vi "XYPlotterUI.vi"() -> ()   [LabVIEW 2025, in "XY Plotter.lvlib" / "XY Plotter.lvclass"]
uses:
  XY Plotter.lvclass
  Users/Public/Documents/Sandia National Labs/TSS Plugin/CEF.lvlibp/Node/mainQref.ctl
  Users/Public/Documents/Sandia National Labs/TSS Plugin/CEF.lvlibp/Node/UserEventRef.ctl
  XY Plotter configuration/XY Plotter.ctl
  Users/Public/Documents/Sandia National Labs/TSS Plugin/CEF.lvlibp/Node/NodeRef.ctl
  Users/Public/Documents/Sandia National Labs/TSS Plugin/CEF.lvlibp/Node/CEF_Node.lvclass
  XY Plotter.lvclass/XY Plotter.ctl
  XY Plotter configuration/XY Plotter configuration.lvclass/XY Plotter configuration.ctl
  <vilib>/Utility/miscctls.llb/LVAnnotationListTypeDef.ctl
  XY Plotter configuration/Read XY Plotter.vi
  XY Plotter configuration/Write XY Plotter.vi
  <vilib>/Analysis/baseanly.llb/Mean (DBL).vi
  C:/Users/Public/Documents/Sandia National Labs/TSS Plugin/CEF.lvlibp/serializable node/CEF_serializable node.lvclass
  C:/Users/Public/Documents/Sandia National Labs/TSS Plugin/CEF.lvlibp/Node/CEF_Node.lvclass
  C:/Working copy/TS Manager/Plugin/Special Test/XY Plotter/XY  Plotter/XY Plotter.lvclass
  <vilib>/Analysis/NI_AALBase.lvlib
  XY Plotter configuration/XY Plotter configuration.lvclass
panel:
  in  "node ref":T1
  in  "XY Plotter Setting":T2={"Data Rate"=100, "Y-Scales"=[{"Label"="Amplitude", "Max"=5.0, "Min"=-5.0, "Unit"=enum."V", "Visible"=TRUE}, {"Label"="", "Max"=100.0, "Min"=-100.0, "Unit"=enum."V", "Visible"=TRUE}], "Note"="", "History Length"=5, "DataLog Path"=path "C:/_Data_Log", "Plot type"=FALSE, "X-Scales"=[{"Label"="Amplitude", "Max"=5.0, "Min"=-5.0, "Unit"=enum."in", "Visible"=TRUE}, {"Label"="", "Max"=100.0, "Min"=-100.0, "Unit"=enum."---", "Visible"=TRUE}], "Plot List"=[{"Plot Name"="Ch1", "X Scale Index"=0, "Y Scale Index"=0, "Visible"=TRUE}, {"Plot Name"="Ch1", "X Scale Index"=0, "Y Scale Index"=0, "Visible"=TRUE}]}
  in  "main queue":T3
  in  "user event":T4
  out "Note":string="ASDFASD\nASDFASD\nF\nASDF\nA\nSDF"
  in  "XY Plot":cluster{"Wavenumber":dbl[], "Data":dbl[]}[](graph)
  in  "Running":bool
  in  "Snap plot":u16(ring)=1 items=["Ch1", "Ch1"]
  in  "Cursor":bool caption="Draw"
  out "Live Loop":u32 caption="ms"
  in  "Settings":bool
  in  "P/N :":string="1D8674-P0100" caption="live data"
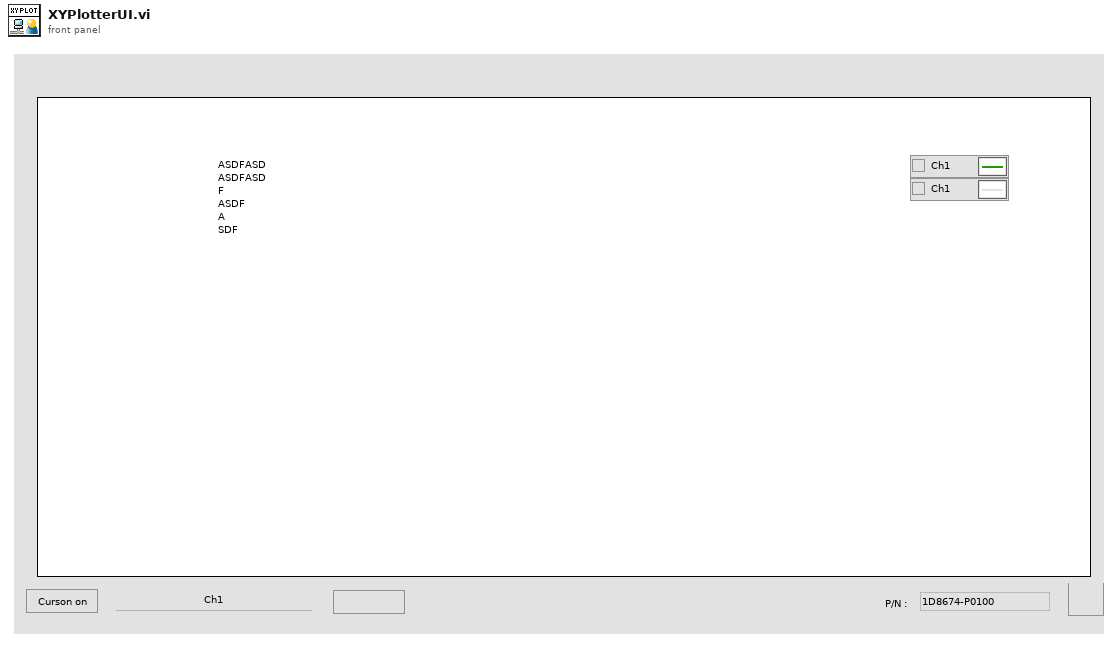
[diagram p1: front panel]
types:
  T1 = typedef "CEF.lvlibp/CEF_Node.lvclass/NodeRef.ctl" = refnum<data-value>
  T2 = typedef "XY Plotter.lvlib/XY Plotter configuration.lvclass/XY Plotter.ctl" = cluster{"Data Rate":i32, "Y-Scales":cluster{"Label":string, "Max":dbl, "Min":dbl, "Unit":enum16{"---", "V", "mA", "sec", "dB", "deg", "in/s", "in", "lbf", "Hz", "psi", "gpm"}, "Visible":bool}[], "Note":string, "History Length":i32, "DataLog Path":path, "Plot type":bool, "X-Scales":cluster{"Label":string, "Max":dbl, "Min":dbl, "Unit":enum16{"---", "V", "mA", "sec", "dB", "deg", "in/s", "in", "lbf", "Hz", "psi", "gpm"}, "Visible":bool}[], "Plot List":cluster{"Plot Name":string, "X Scale Index":u32, "Y Scale Index":u32, "Visible":bool}[]}
  T3 = typedef "CEF.lvlibp/CEF_Node.lvclass/mainQref.ctl" = refnum<queue>
  T4 = typedef "CEF.lvlibp/CEF_Node.lvclass/UserEventRef.ctl" = refnum<user-event>
  T5 = cluster{"XY Plot":refnum<vi>, "Snap plot":refnum<vi>}
  T6 = enum8{"Enabled", "Disabled", "Disabled and Grayed Out"}
  T7 = typedef "LVAnnotationListTypeDef.ctl" = cluster{"Name":string, "Color":u32, "Style":u8, "Point Style":u8, "Name Visible":bool, "Allow Drag":bool, "Annotation Mode":u32, "Plot":i32, "Index":i32, "Position":cluster{"X":dbl, "Y":dbl}, "X Scale":u32, "Y Scale":u32, "Show Arrow":bool, "Lock Name":bool, "Plot Area":i32, "Label Offset":cluster{"X":dbl, "Y":dbl}}[]
  T8 = cluster{"XY Plot":refnum<vi>, "XY Plotter Setting":refnum<vi>, "CursRef":refnum<vi>}
  T9 = typedef "LVPoint32TypeDef.ctl" = cluster{"Horizontal":i32, "Vertical":i32}
  T10 = typedef "LVCursorListTypeDef.ctl" = cluster{"Name":string, "Color":u32, "Style":u8, "Point Style":u8, "Name Visible":bool, "Allow Drag":bool, "Cursor Mode":u32, "Plot":i32, "Index":i32, "Position":cluster{"X":dbl, "Y":dbl}, "X Scale":u32, "Y Scale":u32, "Watch Plots":i32[], "Watch All Plots":bool, "Plot Area":i32, "Label Offset":cluster{"X":dbl, "Y":dbl}}[]
  T11 = cluster{"Plot Name":string, "X Scale Index":u32, "Y Scale Index":u32, "Visible":bool}[]
  T12 = cluster{"Name":string, "Color":u32, "Style":u8, "Point Style":u8, "Name Visible":bool, "Allow Drag":bool, "Annotation Mode":u32, "Plot":i32, "Index":i32, "Position":cluster{"X":dbl, "Y":dbl}, "X Scale":u32, "Y Scale":u32, "Show Arrow":bool, "Lock Name":bool, "Plot Area":i32, "Label Offset":cluster{"X":dbl, "Y":dbl}}
  T13 = cluster{"Shift":bool, "Ctrl":bool, "Alt":bool, "Cmd":bool, "Opt":bool}
  T14 = typedef "eventvkey.ctl" = enum16{"ASCII", "Enter", "Return", "Shift", "Ctrl", "Alt", "Cmd", "Opt", "Caps", "NumLock", "Clear", "Break", "Up", "Down", "Left", "Right", "Insert", "Delete", "Home", "End", "PageUp", "PageDown", "Escape", "Help", "Pause", "ScrollLock", "F1", "F2", "F3", "F4", "F5", "F6", "F7", "F8", "F9", "F10", "F11", "F12", "F13", "F14", "F15", "F16", "F17", "F18", "F19", "F20", "F21", "F22", "F23", "F24", "Play", "VolumeUp", "VolumeDown", "Mute", "Two Byte Char"}
  T15 = cluster{"Running":refnum<vi>, "XY Plot":refnum<vi>, "Snap plot":refnum<vi>}
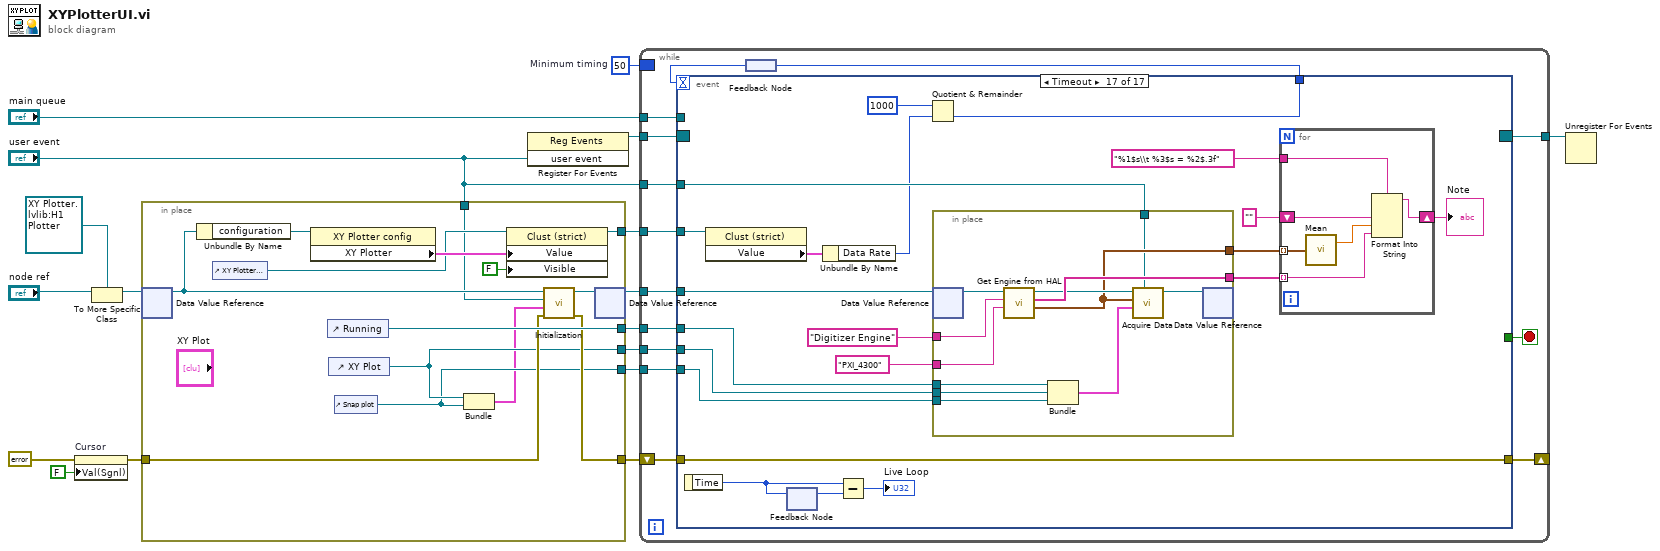
[diagram p0: block diagram]
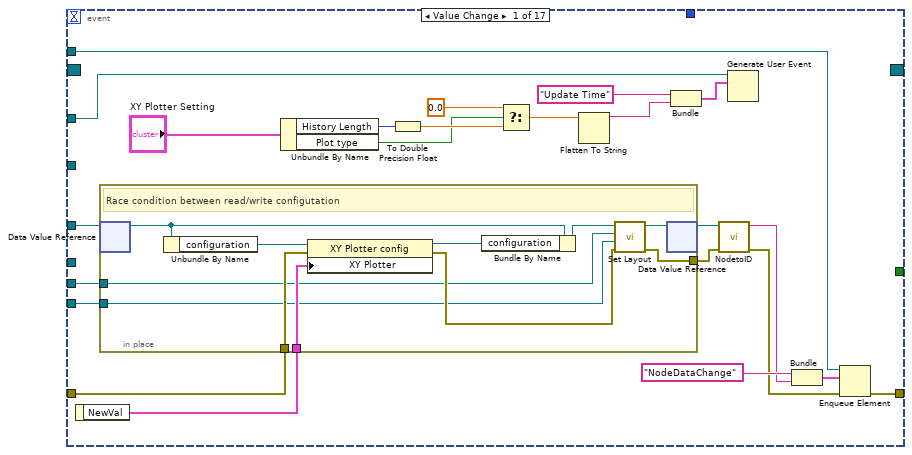
[diagram p2: hidden frame]
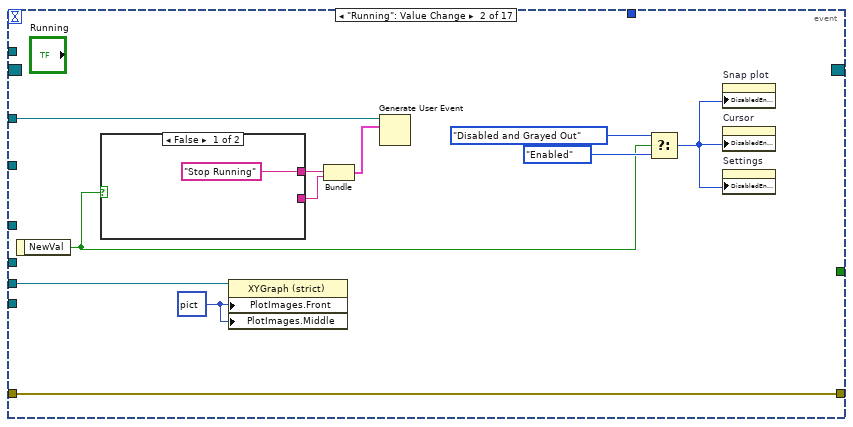
[diagram p3: hidden frame]
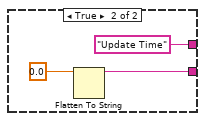
[diagram p4: hidden frame]
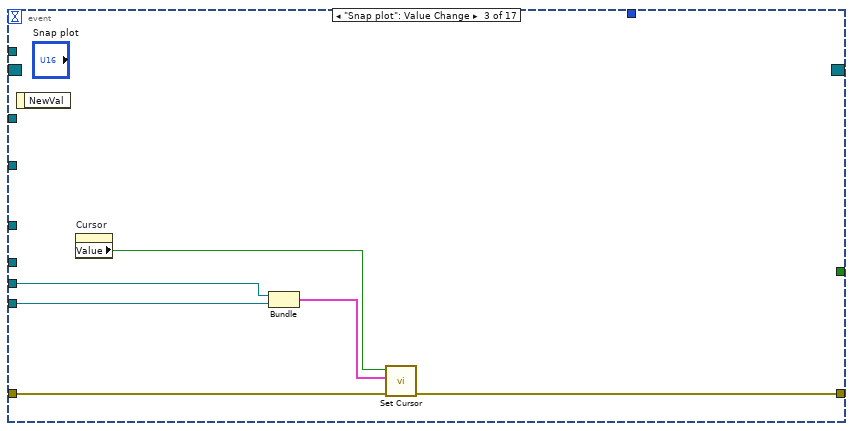
[diagram p5: hidden frame]
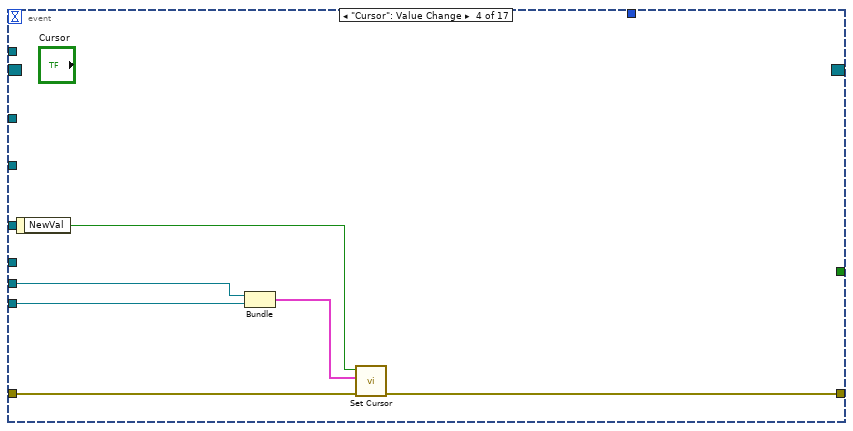
[diagram p6: hidden frame]
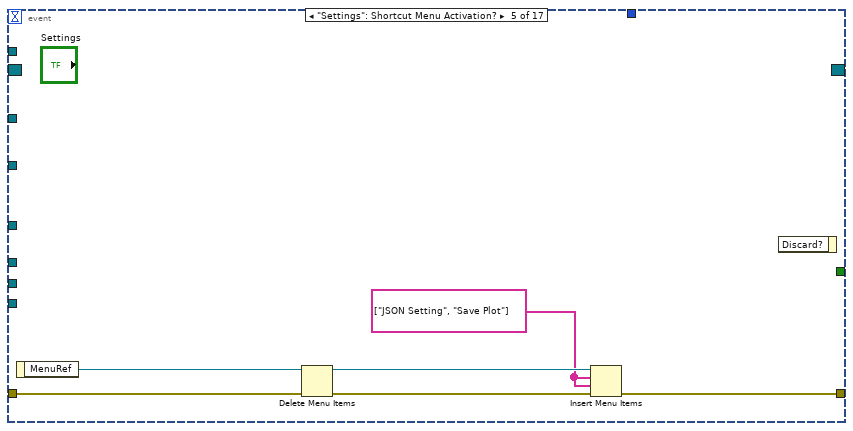
[diagram p7: hidden frame]
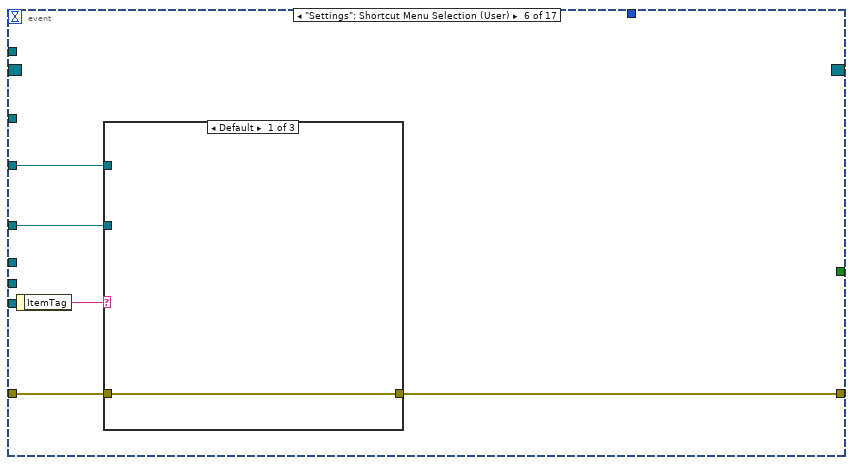
[diagram p8: hidden frame]
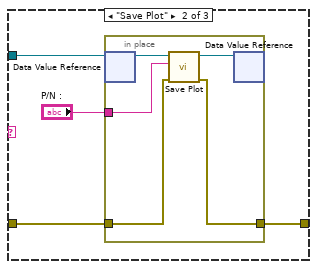
[diagram p9: hidden frame]
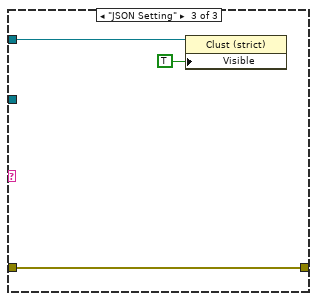
[diagram p10: hidden frame]
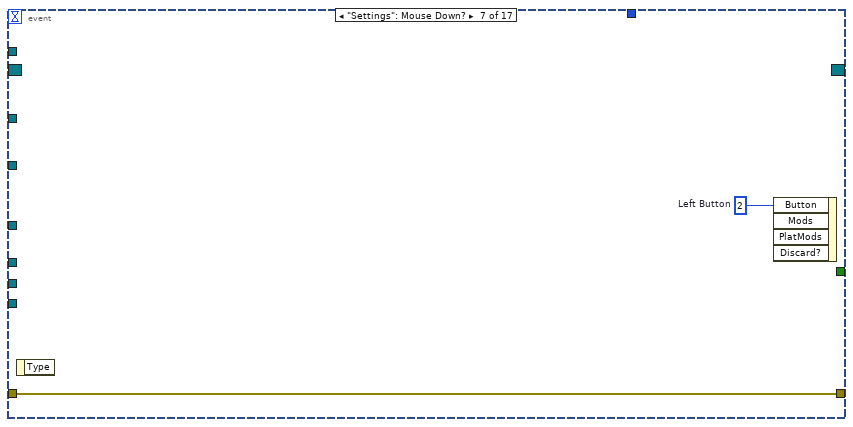
[diagram p11: hidden frame]
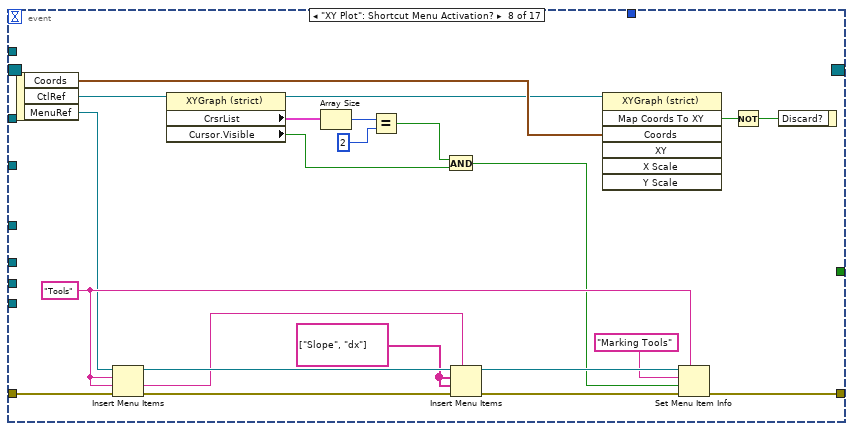
[diagram p12: hidden frame]
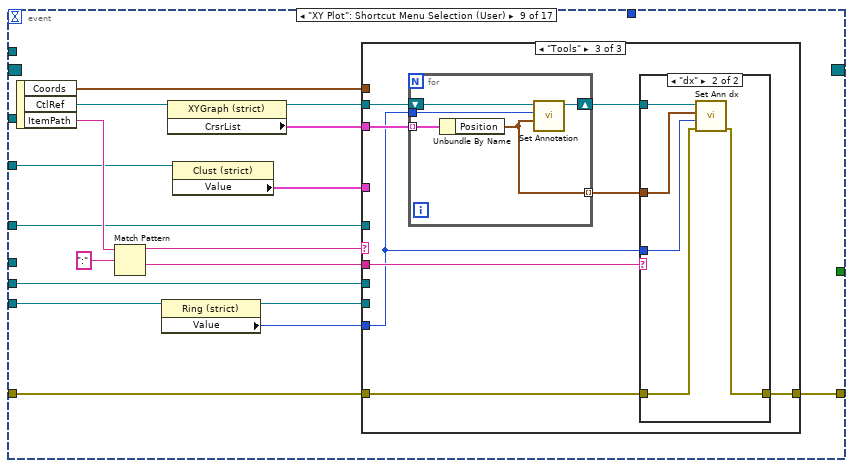
[diagram p13: hidden frame]
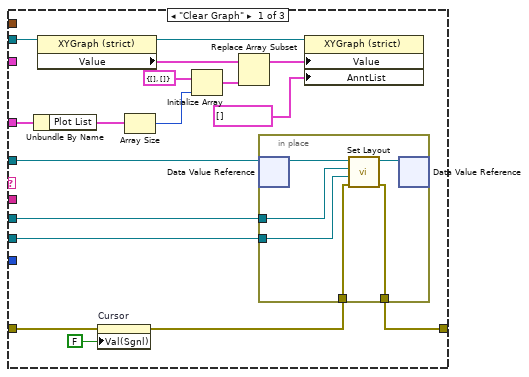
[diagram p14: hidden frame]
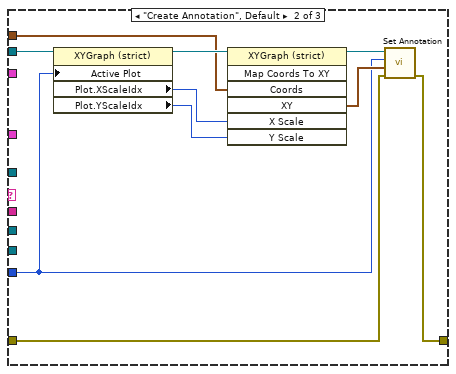
[diagram p15: hidden frame]
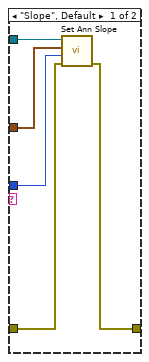
[diagram p16: hidden frame]
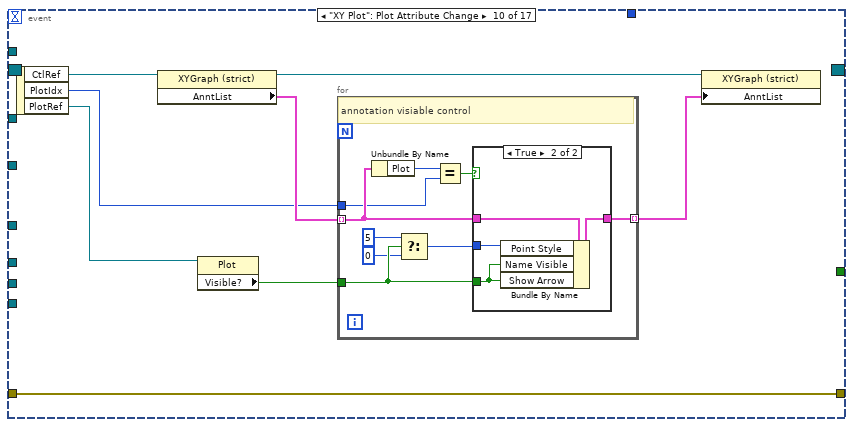
[diagram p17: hidden frame]
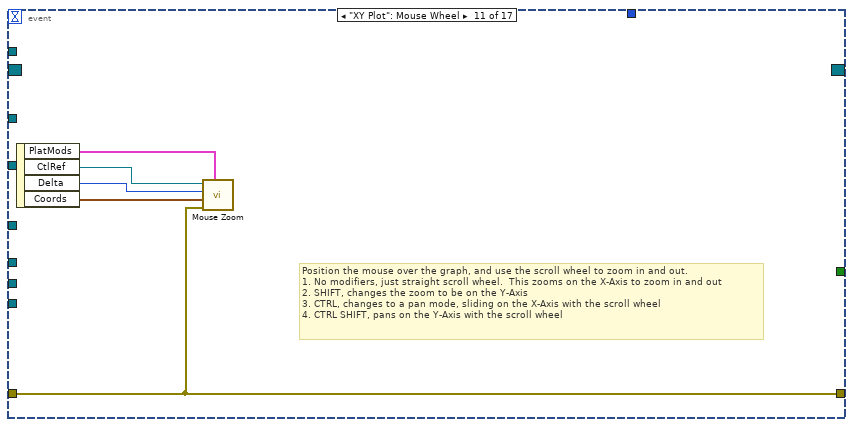
[diagram p19: hidden frame]
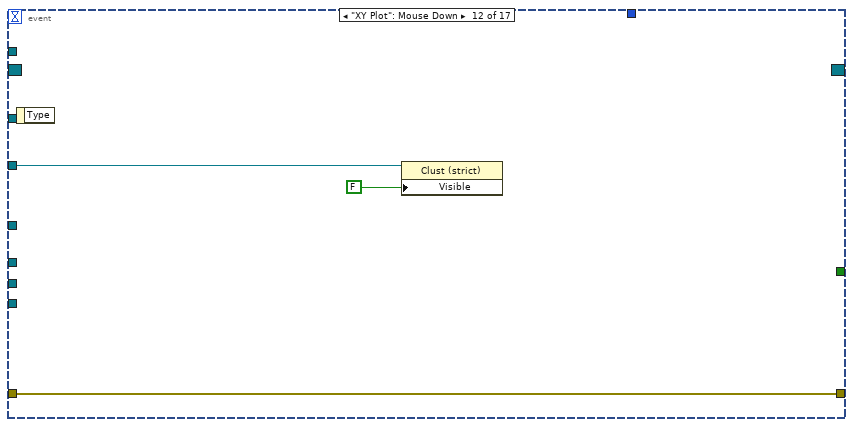
[diagram p20: hidden frame]
diagram:
  w17 = 50  # Minimum timing
  n1 = property on="Cursor" class="Bool (strict)"(error in=errorcluster {"status"=FALSE, "code"=0, "source"=""} ("error in (no error)"), "Val(Sgnl)"=FALSE ("Value (Signaling)")) -> (error out=w2:errorcluster)  [unwired: 1 in, 1 out]
  n2 = To More Specific Class(target class=refnum<data-value> refnum ("data value reference"), reference="node ref") -> (specific class reference=w6:refnum<data-value>)  [unwired: 1 in, 1 out]
  n3 = in-place {
    in-place-border: [w30] -> w12
    in-place-border: [w27] -> w11
    in-place-border: [w20] -> w10
    in-place-border: [w19] -> w9
    in-place-border: [w24] -> w8
    in-place-border: w2 -> [w22]
    in-place-border: "user event" -> [w23]
    n4 = in-place-dvr #1(w6) -> (w26:refnum<class "XY Plotter.lvclass">)  [unwired: 1 out]
    n5 = Unbundle By Name(w26) -> ("configuration"=w31:refnum<class "XY Plotter configuration.lvclass">)
    n6 = control-ref of="XY Plotter Setting"() -> (w28:refnum<vi>)
    n7 = property class="XY Plotter config"(reference=w31) -> ("XY Plotter"=w29:T2)  [unwired: 1 in, 2 out]
    n8 = control-ref of="Running"() -> (w27:refnum<vi>)
    n9 = control-ref of="XY Plot"() -> (w20:refnum<vi>)
    n10 = control-ref of="Snap plot"() -> (w19:refnum<vi>)
    n11 = Bundle("XY Plot"=w20, "Snap plot"=w19) -> (w18:T5)  [unwired: 1 in]
    n12 = property class="Clust (strict)"(reference=w28, "Value"=w29, "Visible"=FALSE) -> (reference out=w30:refnum<vi>)  [unwired: 1 in, 1 out]
    n13 = call-dynamic "Initialization.vi"("error in"=w22, "UI Refs"=w18, "user event"=w23, "XY Plotter"=w26) -> ("error out"=w24:errorcluster, "XY Plotter out"=w25:refnum<class "XY Plotter.lvclass">)  [unwired: 6 in]
    n14 = in-place-dvr #1(w25) -> (w13:refnum<data-value>)  [unwired: 1 out]
  }
  n15 = register-events("user event") -> (reference out=w16:refnum<event-registration>)  [unwired: 2 in, 1 out]
  n16 = while {
    tunnel: [w45] -> w15
    border: w17 -> [_]
    tunnel: w16 -> [w44]
    tunnel: "main queue" -> [w42]
    tunnel: w13 -> [w41]
    tunnel: w12 -> [w39]
    tunnel: w11 -> [w38]
    tunnel: w10 -> [w37]
    tunnel: w9 -> [w36]
    shift-right: [w34] -> _
    shift-left: w8 -> [w35]
    tunnel: "user event" -> [w32]
    stop <- w40 stop-if-true
    n17 = feedback #2() -> (w33:i32)
    n18 = event shown="[16] Timeout" {
      selector: w44 -> [_ _ _ _ _ _ _ _ _ _ _ _ _ _ _ _ _]
      dyn-events: [_ _ _ _ _ _ _ _ _ _ _ _ _ _ _ _ _] -> w45
      timeout: w33 -> [_ _ _ _ _ _ _ _ _ _ _ _ _ _ _ _ _]
      tunnel: [_ _ _ _ _ _ _ _ _ _ _ _ _ _ _ _ w334] -> w43
      tunnel: w42 -> [w63 _ _ _ _ _ _ _ _ _ _ _ _ _ _ _ _]
      tunnel: w41 -> [w68 _ _ _ _ w116 _ _ w162 _ _ _ _ _ w276 _ w346]
      tunnel: [_ _ _ _ _ _ _ _ _ _ _ _ _ _ w283 TRUE _] -> w40
      tunnel: w39 -> [_ _ _ _ _ w114 _ _ w161 _ _ w256 w258 _ _ _ w338]
      tunnel: w38 -> [_ _ _ _ _ _ _ _ _ _ _ _ _ w269 w278 w325 w330]
      tunnel: w37 -> [w47 w87 w96 w103 _ _ _ _ w155 _ _ _ _ _ w277 _ w331]
      tunnel: w36 -> [w46 _ w97 w102 _ _ _ _ w160 _ _ _ w264 _ w275 _ w332]
      tunnel: w35 -> [w58 w86 w100 w106 w109 w115 w131 w136 w157 w228 w250 w255 w262 w268 w280 w324 w347]
      tunnel: [w61 w86 w99 w105 w107 w113 w131 w133 w156 w228 w250 w255 w261 w268 w279 w324 w347] -> w34
      tunnel: w32 -> [w51 w85 _ _ _ _ _ _ _ _ _ _ _ _ _ _ w339]
      event Value Change {
        n19 = event-data() -> ("NewVal"=w59:T2)  [unwired: 1 in]
        n20 = in-place {
          in-place-border: [w71] -> w60
          in-place-border: w59 -> [w77]
          in-place-border: w58 -> [w76]
          in-place-border: w47 -> [w70]
          in-place-border: w46 -> [w69]
          # "Race condition between read/write configutation"
          n21 = in-place-dvr #3(w68) -> (w75:refnum<class "XY Plotter.lvclass">)  [unwired: 1 out]
          n22 = Unbundle By Name(w75) -> ("configuration"=w79:refnum<class "XY Plotter configuration.lvclass">)
          n23 = property class="XY Plotter config"(reference=w79, error in=w76, "XY Plotter"=w77) -> (reference out=w78:refnum<class "XY Plotter configuration.lvclass">, error out=w72:errorcluster)
          n24 = Bundle By Name(cluster=w75, "configuration"=w78) -> (w74:refnum<class "XY Plotter.lvclass">)
          n25 = call "Set Layout.vi"("error in (no error)"=w72, "Snap plot"=w69, "XY Plot"=w70, "XY Plotter"=w74) -> ("error out"=w71:errorcluster, "XY Plotter out"=w73:refnum<class "XY Plotter.lvclass">)  [unwired: 6 in]
          n26 = in-place-dvr #3(w73) -> (w67:refnum<data-value>)  [unwired: 1 out]
        }
        n27 = Unbundle By Name("XY Plotter Setting") -> ("History Length"=w49:i32, "Plot type"=w48:bool)
        n28 = To Double Precision Float(number=w49) -> (double precision float=w54:dbl)
        n29 = Select(t=0.0 ("f"), s=w48, f=w54) -> (s? t:f=w55:dbl)
        n30 = Flatten To String(anything=w55) -> (data string=w56:string)  [unwired: 3 in, 2 out]
        n31 = Bundle("message"="Update Time", "data string"=w56) -> (w57:cluster{"message":string, "data string":string})  [unwired: 1 in]
        n32 = call "NodetoID.vi"("error in"=w60, "node ref"=w67) -> ("error out"=w62:errorcluster, "ID"=w64:string)  [unwired: 8 in]
        n33 = Generate User Event(user event=w51, event data cluster=w57) -> ()  [unwired: 2 in, 2 out]
        n34 = Bundle("Message Name"="NodeDataChange", "ID"=w64) -> (w65:cluster{"Message Name":string, "ID":string})  [unwired: 1 in]
        n35 = Enqueue Element(queue=w63, element=w65, error in (no error)=w62) -> (error out=w61:errorcluster)  [unwired: 1 in, 2 out]
      }
      event "Running": Value Change {
        w80 = picture data[5B] ("Plot Images:Middle")
        n36 = event-data() -> ("NewVal"=w84:bool)  [unwired: 1 in]
        n37 = case shown="False" w84 {
          tunnel: ["Stop Running" ("message") "Update Time" ("message")] -> w82
          tunnel: [_ w92] -> w81
          frame False {
          }
          frame True {
            n38 = Flatten To String(anything=0.0) -> (data string=w92:string)  [unwired: 3 in, 2 out]
          }
        }
        n39 = property class="XYGraph (strict)"(reference=w87, "PlotImages.Front"=w80, "PlotImages.Middle"=w80) -> ()  [unwired: 1 in, 2 out]
        n40 = Bundle("message"=w82, "data string"=w81) -> (w83:cluster{"message":string, "data string":string})  [unwired: 1 in]
        n41 = Generate User Event(user event=w85, event data cluster=w83) -> ()  [unwired: 2 in, 2 out]
        n42 = Select(t=T6."Disabled and Grayed Out" ("Disabled"), s=w84, f=T6."Enabled" ("Disabled")) -> (s? t:f=w88:T6)
        n43 = property on="Snap plot" class="Ring (strict)"("DisabledEnum"=w88) -> ()  [unwired: 2 in, 2 out]
        n44 = property on="Cursor" class="Bool (strict)"("DisabledEnum"=w88) -> ()  [unwired: 2 in, 2 out]
        n45 = property on="Settings" class="Bool"("DisabledEnum"=w88) -> ()  [unwired: 2 in, 2 out]
      }
      event "Snap plot": Value Change {
        n46 = event-data() -> ()  [unwired: 1 in, 1 out]
        n47 = property on="Cursor" class="Bool (strict)"() -> ("Value"=w98:bool)  [unwired: 2 in, 2 out]
        n48 = Bundle("XY Plot"=w96, "Snap plot"=w97) -> (w95:T5)  [unwired: 1 in]
        n49 = call "Set Cursor.vi"("error in (no error)"=w100, "UI Refs"=w95, "Visible(F)"=w98) -> ("error out"=w99:errorcluster)  [unwired: 8 in]
      }
      event "Cursor": Value Change {
        n50 = event-data() -> ("NewVal"=w104:bool)  [unwired: 1 in]
        n51 = Bundle("XY Plot"=w103, "Snap plot"=w102) -> (w101:T5)  [unwired: 1 in]
        n52 = call "Set Cursor.vi"("error in (no error)"=w106, "UI Refs"=w101, "Visible(F)"=w104) -> ("error out"=w105:errorcluster)  [unwired: 8 in]
      }
      event "Settings": Shortcut Menu Activation? {
        w110 = string[] ["JSON Setting", "Save Plot"] ("item names")
        n53 = event-data() -> ("MenuRef"=w112:refnum<k9>)  [unwired: 1 in]
        n54 = Delete Menu Items(6:w109, 9:w112) -> (0:w108:errorcluster, 3:w111:refnum<k9>)  [unwired: 2 in]
        n55 = Insert Menu Items(6:w108, 7:w110, 8:w110, 9:w111) -> (0:w107:errorcluster)  [unwired: 2 in, 2 out]
        n56 = event-data() -> ()  [unwired: 2 in, 1 out]
      }
      event "Settings": Shortcut Menu Selection (User) {
        n57 = event-data() -> ("ItemTag"=w117:string)  [unwired: 1 in]
        n58 = case shown="Default" w117 {
          tunnel: w116 -> [_ w121 _]
          tunnel: w115 -> [w118 w120 w130]
          tunnel: [w118 w119 w130] -> w113
          tunnel: w114 -> [_ _ w129]
          frame Default {
          }
          frame "Save Plot" {
            n59 = in-place {
              in-place-border: "P/N :" -> [w127]
              in-place-border: w120 -> [w124]
              in-place-border: [w123] -> w119
              n60 = in-place-dvr #4(w121) -> (w126:refnum<class "XY Plotter.lvclass">)  [unwired: 1 out]
              n61 = call-dynamic "Save Plot.vi"("error in (no error)"=w124, "Partnumber"=w127, "XY Plotter"=w126) -> ("error out"=w123:errorcluster, "XY Plotter out"=w125:refnum<class "XY Plotter.lvclass">)  [unwired: 7 in]
              n62 = in-place-dvr #4(w125) -> ()  [unwired: 2 out]
            }
          }
          frame "JSON Setting" {
            n63 = property class="Clust (strict)"(reference=w129, "Visible"=TRUE) -> ()  [unwired: 1 in, 2 out]
          }
        }
      }
      event "Settings": Mouse Down? {
        w132 = u16 2  # Left Button
        n64 = event-data() -> ()  [unwired: 1 in, 1 out]
        n65 = event-data("Button"=w132) -> ()  [unwired: 4 in, 1 out]
      }
      event "XY Plot": Shortcut Menu Activation? {
        w149 = string[] ["Slope", "dx"]
        w148 = "Tools"
        n66 = event-data() -> ("Coords"=w147:T9, "CtlRef"=w143:refnum<vi>, "MenuRef"=w144:refnum<k9>)  [unwired: 1 in]
        n67 = Insert Menu Items(6:w136, 7:w148, 8:w148, 9:w144) -> (0:w135:errorcluster, 1:w151:string, 3:w152:refnum<k9>)  [unwired: 2 in]
        n68 = property class="XYGraph (strict)"(reference=w143) -> (reference out=w145:refnum<vi>, "CrsrList"=w140:T10, "Cursor.Visible"=w137:bool)  [unwired: 1 in, 1 out]
        n69 = Array Size(array=w140) -> (size(s)=w142:i32)
        n70 = Equal?(x=w142, y=2) -> (x = y?=w138:bool)
        n71 = And(x=w138, y=w137) -> (x .and. y?=w139:bool)
        n72 = Insert Menu Items(5:w151, 6:w135, 7:w149, 8:w149, 9:w152) -> (0:w134:errorcluster, 3:w150:refnum<k9>)  [unwired: 1 in, 1 out]
        n73 = invoke class="XYGraph (strict)" method="Map Coords To XY"(reference=w145, "Coords"=w147) -> ("Map Coords To XY"=w154:bool)  [unwired: 5 in, 6 out]
        n74 = Set Menu Item Info(7:w148, 8:w134, 9:w139, 10:"Marking Tools" ("item name"), 11:w150) -> (0:w133:errorcluster)  [unwired: 2 in, 1 out]
        n75 = Not(x=w154) -> (.not. x?=w153:bool)
        n76 = event-data("Discard?"=w153) -> ()  [unwired: 1 in, 1 out]
      }
      event "XY Plot": Shortcut Menu Selection (User) {
        n77 = event-data() -> ("Coords"=w164:T9, "CtlRef"=w165:refnum<vi>, "ItemPath"=w170:string)  [unwired: 1 in]
        n78 = Match Pattern(string=w170, regular expression=":") -> (before substring=w168:string, after substring=w169:string)  [unwired: 1 in, 2 out]
        n79 = property class="Ring (strict)"(reference=w160) -> (reference out=w158:refnum<vi>, "Value"=w159:u16)  [unwired: 1 in, 1 out]
        n80 = property class="XYGraph (strict)"(reference=w165) -> (reference out=w167:refnum<vi>, "CrsrList"=w166:T10)  [unwired: 1 in, 1 out]
        n81 = property class="Clust (strict)"(reference=w161) -> ("Value"=w163:T2)  [unwired: 1 in, 2 out]
        n82 = case shown="\"Tools\"" w168 {
          tunnel: w167 -> [w188 w203 w210]
          tunnel: w169 -> [_ _ w212]
          tunnel: w166 -> [_ _ w211]
          tunnel: w164 -> [_ w198 _]
          tunnel: w159 -> [_ w197 w207]
          tunnel: w163 -> [w180 _ _]
          tunnel: w162 -> [w177 _ _]
          tunnel: w158 -> [w176 _ _]
          tunnel: w157 -> [w175 w196 w206]
          tunnel: [w173 w195 w205] -> w156
          tunnel: w155 -> [w172 _ _]
          frame "Clear Graph" {
            n83 = Unbundle By Name(w180) -> ("Plot List"=w179:T11)
            n84 = property class="XYGraph (strict)"(reference=w188) -> (reference out=w186:refnum<vi>, "Value"=w183:cluster{"Wavenumber":dbl[], "Data":dbl[]}[])  [unwired: 1 in, 1 out]
            n85 = property on="Cursor" class="Bool (strict)"(error in=w175, "Val(Sgnl)"=FALSE ("Value (Signaling)")) -> (error out=w174:errorcluster)  [unwired: 1 in, 1 out]
            n86 = Array Size(array=w179) -> (size(s)=w178:i32)
            n87 = Initialize Array(cluster{"Wavenumber":dbl[], "Data":dbl[]} {"Wavenumber"=[], "Data"=[]} ("Spectrum"), w178) -> (w184:cluster{"Wavenumber":dbl[], "Data":dbl[]}[])
            n88 = Replace Array Subset(array=w183, new element=w184) -> (w182:cluster{"Wavenumber":dbl[], "Data":dbl[]}[])  [unwired: 1 in]
            n89 = in-place {
              in-place-border: w176 -> [w189]
              in-place-border: w174 -> [w192]
              in-place-border: [w191] -> w173
              in-place-border: w172 -> [w190]
              n90 = in-place-dvr #5(w177) -> (w194:refnum<class "XY Plotter.lvclass">)  [unwired: 1 out]
              n91 = call "Set Layout.vi"("error in (no error)"=w192, "Snap plot"=w189, "XY Plot"=w190, "XY Plotter"=w194) -> ("error out"=w191:errorcluster, "XY Plotter out"=w193:refnum<class "XY Plotter.lvclass">)  [unwired: 6 in]
              n92 = in-place-dvr #5(w193) -> ()  [unwired: 2 out]
            }
            n93 = property class="XYGraph (strict)"(reference=w186, "Value"=w182, "AnntList"=T7 [] ("Annotation List")) -> ()  [unwired: 1 in, 2 out]
          }
          frame "Create Annotation", Default {
            n94 = property class="XYGraph (strict)"(reference=w203, "Active Plot"=w197) -> (reference out=w204:refnum<vi>, "Plot.XScaleIdx"=w200:u32, "Plot.YScaleIdx"=w199:u32)  [unwired: 1 in, 1 out]
            n95 = invoke class="XYGraph (strict)" method="Map Coords To XY"(reference=w204, "Coords"=w198, "X Scale"=w200, "Y Scale"=w199) -> (reference out=w202:refnum<vi>, "XY"=w201:cluster{"X":dbl, "Y":dbl})  [unwired: 3 in, 5 out]
            n96 = call "Set Annotation.vi"("error in"=w196, "XY Position"=w201, "Active Plot"=w197, "XY Plot"=w202) -> ("error out"=w195:errorcluster)  [unwired: 6 in, 1 out]
          }
          frame "Tools" {
            n97 = for {
              tunnel: w207 -> [w214]
              tunnel: w211 -> [w217] mode=indexing
              tunnel: [w213] -> w209 mode=indexing
              shift-right: [w215] -> w208
              shift-left: w210 -> [w216]
              n98 = Unbundle By Name(w217) -> ("Position"=w213:cluster{"X":dbl, "Y":dbl})
              n99 = call "Set Annotation.vi"("XY Position"=w213, "Active Plot"=w214, "XY Plot"=w216) -> ("XY Plot out"=w215:refnum<vi>)  [unwired: 7 in, 1 out]
            }
            n100 = case shown="\"dx\"" w212 {
              tunnel: w209 -> [w221 w226]
              tunnel: w208 -> [w222 w227]
              tunnel: w207 -> [w220 w225]
              tunnel: w206 -> [w219 w224]
              tunnel: [w218 w223] -> w205
              frame "Slope", Default {
                n101 = call "Set Ann Slope.vi"("error in"=w219, "Active Plot"=w220, "Points"=w221, "XY Plot"=w222) -> ("error out"=w218:errorcluster)  [unwired: 6 in, 1 out]
              }
              frame "dx" {
                n102 = call "Set Ann dx.vi"("error in"=w224, "Active Plot"=w225, "Points"=w226, "XY Plot"=w227) -> ("error out"=w223:errorcluster)  [unwired: 6 in, 1 out]
              }
            }
          }
        }
      }
      event "XY Plot": Plot Attribute Change {
        n103 = event-data() -> ("CtlRef"=w235:refnum<vi>, "PlotIdx"=w230:i32, "PlotRef"=w231:refnum<vi>)  [unwired: 1 in]
        n104 = property class="XYGraph (strict)"(reference=w235) -> (reference out=w229:refnum<vi>, "AnntList"=w233:T7)  [unwired: 1 in, 1 out]
        n105 = property class="Plot"(reference=w231) -> ("Visible?"=w232:bool)  [unwired: 1 in, 2 out]
        n106 = for {
          tunnel: w233 -> [w244] mode=indexing
          tunnel: w230 -> [w240]
          tunnel: w232 -> [w242]
          tunnel: [w243] -> w234 mode=indexing
          # "annotation visiable control"
          n107 = Unbundle By Name(w244) -> ("Plot"=w239:i32)
          n108 = Select(t=u8 5 ("Point Style"), s=w242, f=u8 0 ("Point Style")) -> (s? t:f=w236:u8)
          n109 = Equal?(x=w239, y=w240) -> (x = y?=w241:bool)
          n110 = case shown="True" w241 {
            tunnel: w244 -> [w245 w249]
            tunnel: [w245 w248] -> w243
            tunnel: w242 -> [_ w247]
            tunnel: w236 -> [_ w246]
            frame False {
            }
            frame True {
              n111 = Bundle By Name(cluster=w249, "Point Style"=w246, "Name Visible"=w247, "Show Arrow"=w247) -> (w248:T12)
            }
          }
        }
        n112 = property class="XYGraph (strict)"(reference=w229, "AnntList"=w234) -> ()  [unwired: 1 in, 2 out]
      }
      event "XY Plot": Mouse Wheel {
        # "Position the mouse over the graph, and use the scroll wheel to zoom in and out.  \n1. No modifiers, just straight scroll wheel.  This zooms on the X-Axis to zoom in and out\n2. SHIFT, changes the zoom to be on the Y-Axis\n3. CTRL, changes to a pan mode, sliding on the X-Axis with the scroll wheel\n4. CTRL SHIFT, pans on the Y-Axis with the scroll wheel"
        n113 = event-data() -> ("PlatMods"=w254:T13, "CtlRef"=w251:refnum<vi>, "Delta"=w253:i32, "Coords"=w252:T9)  [unwired: 1 in]
        n114 = call "Mouse Zoom.vi"("PlatMods"=w254, "error in (no error)"=w250, "XY"=w252, "Delta"=w253, "XY Graph"=w251) -> ()  [unwired: 7 in]
      }
      event "XY Plot": Mouse Down {
        n115 = event-data() -> ()  [unwired: 1 in, 1 out]
        n116 = property class="Clust (strict)"(reference=w256, "Visible"=FALSE) -> ()  [unwired: 1 in, 2 out]
      }
      event "XY Plot": Cursor Move {
        n117 = event-data() -> ("CtlRef"=w267:refnum<vi>, "CursRef"=w263:refnum<vi>, "CursLoc"=w266:cluster{"X":dbl, "Y":dbl})  [unwired: 1 in]
        n118 = Bundle By Name(cluster=T8 {"XY Plot"=refnum, "XY Plotter Setting"=refnum, "CursRef"=refnum} ("UI Refs"), "XY Plotter Setting"=w258, "XY Plot"=w267, "CursRef"=w263) -> (w259:T8)
        n119 = property class="Ring (strict)"(reference=w264) -> ("Value"=w265:u16)  [unwired: 1 in, 2 out]
        n120 = call "Cursor Move.vi"("error in (no error)"=w262, "Active Plot"=w265, "CursLocation"=w266, "UI Refs"=w259) -> ("error out"=w261:errorcluster)  [unwired: 7 in]
      }
      event Key Down? {
        n121 = event-data() -> ("VKey"=w270:T14)  [unwired: 1 in]
        n122 = case shown="\"F8\"" w270 {
          tunnel: [_ FALSE ("Discard?") _] -> w271
          tunnel: w269 -> [_ _ w273]
          frame Default {
          }
          frame "F8" {
            # "User Event to control start and stop"
          }
          frame "F4" {
            n123 = property class="Bool (strict)"(reference=w273, "Val(Sgnl)"=FALSE ("Value (Signaling)")) -> ()  [unwired: 1 in, 2 out]
          }
        }
        n124 = event-data("Discard?"=w271) -> ()  [unwired: 1 in, 1 out]
      }
      event User Event {
        n125 = event-data() -> ("command"=w282:string, "data"=w281:string)  [unwired: 1 in]
        n126 = case shown="\"Stop\"" w282 {
          tunnel: [_ _ _ TRUE] -> w283
          tunnel: w281 -> [_ w293 _ _]
          tunnel: w280 -> [w284 w291 w306 w321]
          tunnel: [w284 w285 w310 w321] -> w279
          tunnel: w278 -> [_ w288 _ _]
          tunnel: w277 -> [_ w295 w308 w320]
          tunnel: w276 -> [_ w294 w312 _]
          tunnel: w275 -> [_ w287 w309 _]
          frame Default {
          }
          frame "Run" {
            n127 = Unflatten From String(type=TRUE ("Value (Signaling)"), binary string=w293, error in (no error)=w291) -> (value=w289:bool, error out=w290:errorcluster)  [unwired: 2 in, 1 out]
            n128 = property class="Bool (strict)"(reference=w288, "Val(Sgnl)"=w289) -> ()  [unwired: 1 in, 2 out]
            n129 = property on="Cursor" class="Bool (strict)"(error in=w290, "Val(Sgnl)"=FALSE ("Value (Signaling)")) -> (error out=w286:errorcluster)  [unwired: 1 in, 1 out]
            n130 = case shown="True" w289 {
              tunnel: w295 -> [_ w301]
              tunnel: w294 -> [_ w302]
              tunnel: w287 -> [_ w300]
              tunnel: w286 -> [w297 w298]
              tunnel: [w297 w298] -> w285
              frame False {
              }
              frame True {
                n131 = Bundle("XY Plot"=w301, "Snap plot"=w300) -> (w299:T5)  [unwired: 1 in]
                n132 = in-place {
                  in-place-border: w299 -> [w303]
                  n133 = in-place-dvr #6(w302) -> (w305:refnum<class "XY Plotter.lvclass">)  [unwired: 1 out]
                  n134 = call-dynamic "Run.vi"("UI Refs"=w303, "XY Plotter"=w305) -> ("XY Plotter out"=w304:refnum<class "XY Plotter.lvclass">)  [unwired: 8 in, 1 out]
                  n135 = in-place-dvr #6(w304) -> ()  [unwired: 2 out]
                }
              }
            }
          }
          frame "Refresh" {
            n136 = in-place {
              in-place-border: w306 -> [w316]
              in-place-border: [w315] -> w307
              in-place-border: w309 -> [w313]
              in-place-border: w308 -> [w314]
              n137 = in-place-dvr #7(w312) -> (w318:refnum<class "XY Plotter.lvclass">)  [unwired: 1 out]
              n138 = call "Set Layout.vi"("error in (no error)"=w316, "Snap plot"=w313, "XY Plot"=w314, "XY Plotter"=w318) -> ("error out"=w315:errorcluster, "XY Plotter out"=w317:refnum<class "XY Plotter.lvclass">)  [unwired: 6 in]
              n139 = in-place-dvr #7(w317) -> ()  [unwired: 2 out]
            }
            n140 = property on="Cursor" class="Bool (strict)"(error in=w307, "Val(Sgnl)"=FALSE ("Value (Signaling)")) -> (error out=w310:errorcluster)  [unwired: 1 in, 1 out]
          }
          frame "Stop" {
            w319 = picture data[5B] ("Plot Images:Back")
            n141 = property class="XYGraph (strict)"(reference=w320, "PlotImages.Back"=w319, "PlotImages.Front"=w319, "PlotImages.Middle"=w319) -> ()  [unwired: 1 in, 2 out]
          }
        }
      }
      event Panel Close? {
        n142 = event-data() -> ()  [unwired: 1 in, 1 out]
        n143 = property class="Bool (strict)"(reference=w325, "Val(Sgnl)"=FALSE ("Value")) -> ()  [unwired: 1 in, 2 out]
        n144 = disable-structure shown="Default" {
          disable-tunnel: [TRUE ("Discard?") FALSE ("Discard?")] -> w327
          frame condition #0 (active) {
          }
          frame condition #1 {
          }
        }
        n145 = event-data("Discard?"=w327) -> ()  [unwired: 1 in, 1 out]
      }
      event Timeout {
        n146 = event-data() -> ("Time"=w349:u32)  [unwired: 1 in]
        n147 = property class="Clust (strict)"(reference=w338) -> ("Value"=w337:T2)  [unwired: 1 in, 2 out]
        n148 = feedback #8() -> (w350:u32)  [unwired: 1 in]
        n149 = feedback-in #8(w349) -> ()
        n150 = Unbundle By Name(w337) -> ("Data Rate"=w336:i32)
        n151 = Subtract(x=w349, y=w350) -> (x-y=→"Live Loop":u32)
        n152 = Quotient & Remainder(x=1000, y=w336) -> (floor(x/y)=w334:i32)  [unwired: 1 out]
        n153 = in-place {
          in-place-border: [w362] -> w343
          in-place-border: [w367] -> w344
          in-place-border: "Digitizer Engine" ("Engine") -> [w366]
          in-place-border: "PXI_4300" ("Instrument") -> [w365]
          in-place-border: w339 -> [w361]
          in-place-border: w332 -> [w360]
          in-place-border: w331 -> [w359]
          in-place-border: w330 -> [w358]
          n154 = in-place-dvr #9(w346) -> (w368:refnum<class "XY Plotter.lvclass">)  [unwired: 1 out]
          n155 = call "Get Engine from HAL.vi"("Instrument"=w365, "Engine"=w366, "XY Plotter in"=w368) -> ("Waveforms"=w362:waveform(dbl)[], "Channels"=w367:string[], "XY Plotter out"=w364:refnum<class "XY Plotter.lvclass">)  [unwired: 5 in, 1 out]
          n156 = Bundle("Running"=w358, "XY Plot"=w359, "Snap plot"=w360) -> (w357:T15)  [unwired: 1 in]
          n157 = call-dynamic "Acquire Data.vi"("user event"=w361, "UI Refs"=w357, "Waveforms"=w362, "XY Plotter"=w364) -> ("XY Plotter out"=w363:refnum<class "XY Plotter.lvclass">)  [unwired: 6 in, 1 out]
          n158 = in-place-dvr #9(w363) -> ()  [unwired: 2 out]
        }
        n159 = for {
          shift-right: [w355] -> w333
          shift-left: "" ("format string") -> [w356]
          tunnel: w343 -> [w354] mode=indexing
          tunnel: w344 -> [w351] mode=indexing
          tunnel: "%1$s\\t %3$s = %2$.3f" ("format string") -> [w353]
          n160 = call-poly <vilib>:"Mean.vi"("X"=w354) -> ("mean"=w352:dbl)  [unwired: 1 out]
          n161 = Format Into String(format string=w353, w356, w352, w351) -> (resulting string=w355:string)  [unwired: 2 in, 1 out]
        }
        "Note" <- w333
      }
    }
    n162 = feedback-in #2(w43) -> ()
  }
  n163 = Unregister For Events(event registration refnum=w15) -> ()  [unwired: 1 in, 1 out]
